vi "Update Method Setter.vi"(5 "Library":refnum<vi>, 7 "RPC Method Name":string, 8 "error in (no error)":errorcluster, 10 "Response Metadata Name":string, 11 "Server class in":refnum<vi>) -> (0 "error out":errorcluster, 3 "Server class out":refnum<vi>)   [LabVIEW 2019, in "gRPC Template Creation Utility.lvlib"]
uses:
  gRPC Template Creation Utility.lvlib
  TypeDefs/Method Accessor Type.ctl
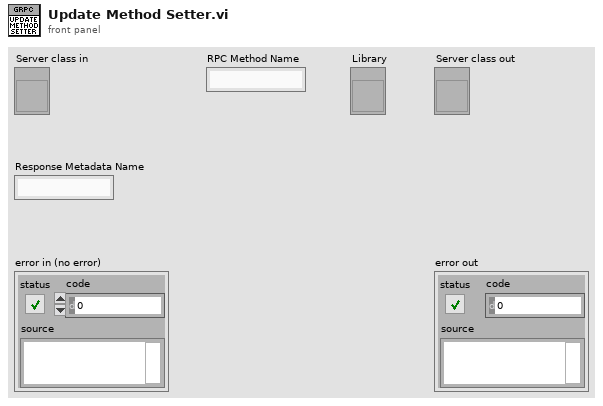
[diagram p1: front panel]
types:
  T1 = typedef "gRPC Template Creation Utility.lvlib/Method Accessor Type.ctl" = string
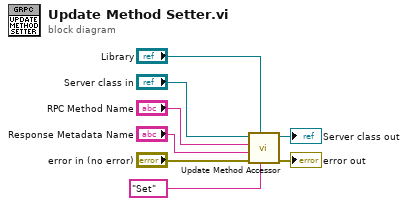
[diagram p0: block diagram]
diagram:
  n1 = call "Update Method Accessor.vi"("accessor type"=T1 "Set", "library"="Library", "error in (no error)"="error in (no error)", "method message metadata name"="Response Metadata Name", "rpc method name"="RPC Method Name", "server class in"="Server class in") -> ("error out"=→"error out":errorcluster, "server class out"=→"Server class out":refnum<vi>)  [unwired: 4 in]
